vi "macro_DCMotor_Pick.vi"   [LabVIEW 2019, in "Trajectory_Library.lvlib"]
uses:
  Trajectory_Library.lvlib
  Enum/DCMOTOR_TYPES_ENUM.ctl
types:
  T1 = typedef "Trajectory_Library.lvlib/DCMOTOR_TYPES_ENUM.ctl" = enum16{"CIM", "AndyMark 9015", "Andy Mark RS 775 125", "Bag", "BaneBots RS 550", "BaneBots RS 775", "Falcon 500", "Mini CIM", "NEO", "NEO 550", "Romi BuiltIn", "Vex 775 Pro", "Snow Blower AM 2235A", "Bosch Seat AM 3493", "Falcon 500 FOC", "Kraken X60", "Kraken X60 FOC", "NEO Vortex"}
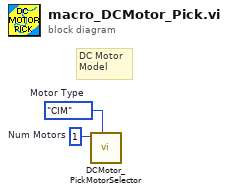
[diagram p0: block diagram]
diagram:
  w1 = 1  # Num Motors
  w2 = DCMOTOR_TYPES_ENUM."CIM"  # Motor Type
  # "DC Motor\nModel"
  n1 = call "DCMotor_PickMotorSelector.vi"("DCMOTOR_TYPES"=w2, "Num Motors"=w1) -> ()  [unwired: 9 in, 1 out]
